vi "D_Close.vi"(8 "error in (no error)":errorcluster, 11 "bIDList":u8[](array[numeric])) -> (0 "error out":errorcluster, 4 "TorF":i32)   [LabVIEW 2017]
uses:
  LabVIEW2018/hpkSLMdaLV.dll
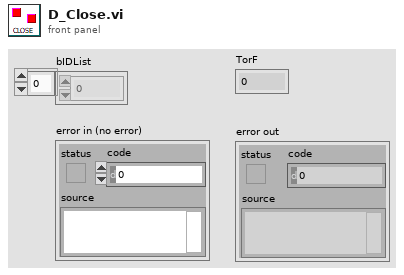
[diagram p1: front panel]
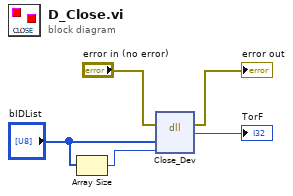
[diagram p0: block diagram]
diagram:
  n1 = Array Size(array="bIDList") -> (size(s)=w2:i32)
  n2 = dll-call lib="C:/Users/hs5921/Desktop/LabVIEW2018/hpkSLMdaLV.dll" fn="Close_Dev"(error in="error in (no error)", "bIDList"="bIDList", "bIDSize"=w2) -> (error out=→"error out":errorcluster, "返り値タイプ"=→"TorF":i32)  [unwired: 4 in, 1 out]
